vi "RFH-convert_folder-r140-2.vi"(5 "Destination Folder":path, 7 "Folder Path":path, 9 "Max Frequency (6G)":dbl=6000000000.0, 10 "Min Frequency  (0.3G)":dbl=300000000.0) -> (0 "error out":errorcluster, 2 "All Good?":bool, 4 "Last Value":T1)   [LabVIEW 2020, in "RFH-Reflection_File_Handler.lvlib"]
doc: "Converts all R140 files of a folder to the common format, on the frequencies of a LibreVNA source file, using RFH-convert_folder-r140."
uses:
  RFH-Reflection_File_Handler.lvlib
  RFH-common_data_format.ctl
panel:
  in  "source":string
  in  "pre-modifier":string="Ref-"
  in  "Xi Source libreVNA":path
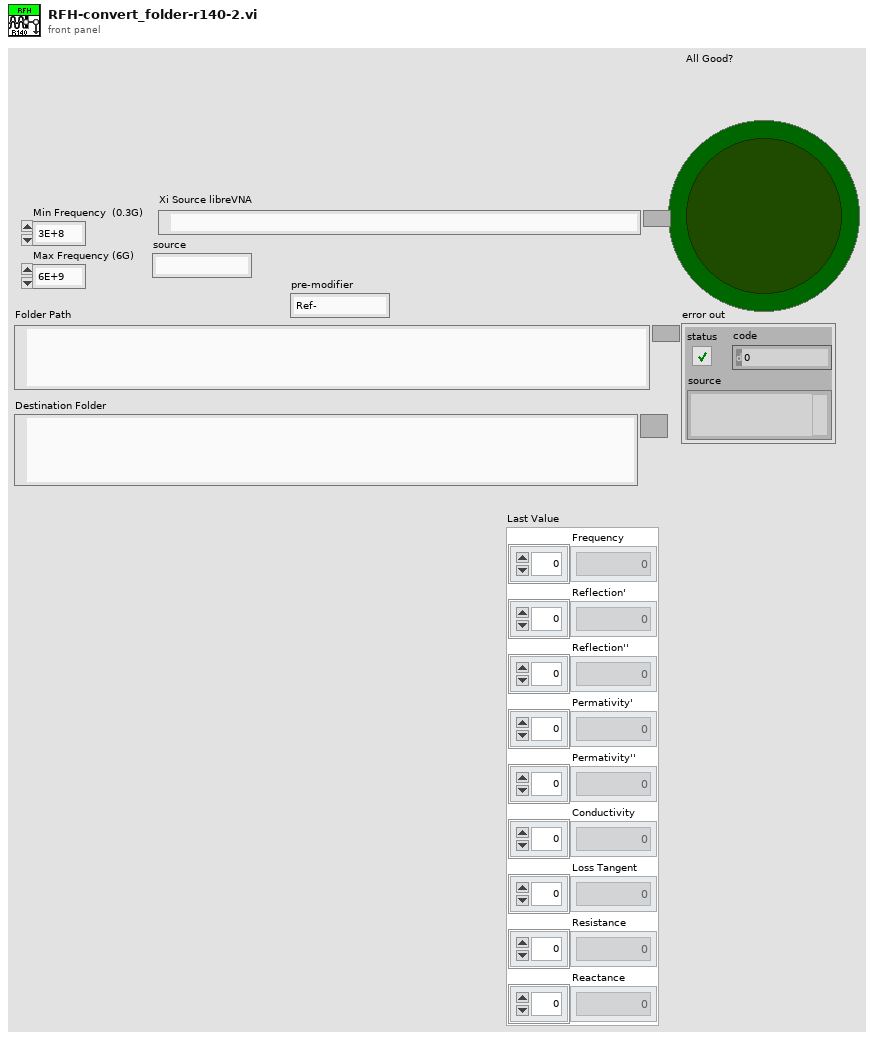
[diagram p1: front panel]
types:
  T1 = typedef "RFH-Reflection_File_Handler.lvlib/RFH-common_data_format.ctl" = cluster{"Frequency":dbl[], "Reflection'":dbl[], "Reflection''":dbl[], "Permativity'":dbl[], "Permativity''":dbl[], "Conductivity":dbl[], "Loss Tangent":dbl[], "Resistance":dbl[], "Reactance":dbl[]}
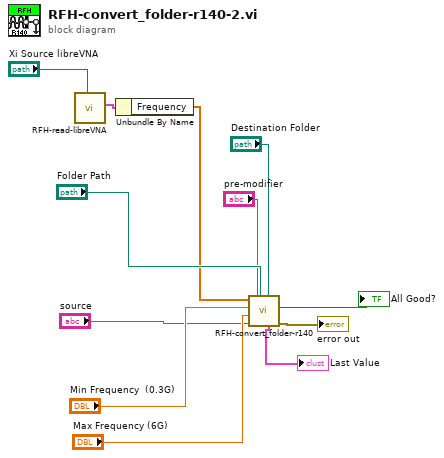
[diagram p0: block diagram]
diagram:
  n1 = call "RFH-read-libreVNA.vi"("file path (dialog if empty)"="Xi Source libreVNA") -> ("Common Format"=w2:T1)  [unwired: 9 in, 1 out]
  n2 = Unbundle By Name(w2) -> ("Frequency"=w10:dbl[])
  n3 = call "RFH-convert_folder-r140.vi"("pre-modifier"="pre-modifier", "Destination Folder"="Destination Folder", "Folder Path"="Folder Path", "source"="source", "Max Frequency (6G)"="Max Frequency (6G)", "Min Frequency  (0.3G)"="Min Frequency  (0.3G)", "Xi"=w10) -> ("error out"=→"error out":errorcluster, "All Good?"=→"All Good?":bool, "Last Value"=→"Last Value":T1)  [unwired: 2 in]
